vi "Digital_Input_Output_Ex.vi"() -> ()   [LabVIEW 2026]
panel:
  in  "Canal Read":u8
  out "Out":bool
  in  "VISA resource name":refnum<visa-resource-name>
  in  "Canal Write":u8
  out "respuesta":string
  in  "Stop Button":bool
  out "error out":errorcluster
  # "Ejemplo: Digital Input Output"
  # "Descripción: Lee un pin digital de entrada y escribe su estado en un pin de salida del microcontrolador."
  # "Configuracion"
  # "Indicadores"
  # "Control"
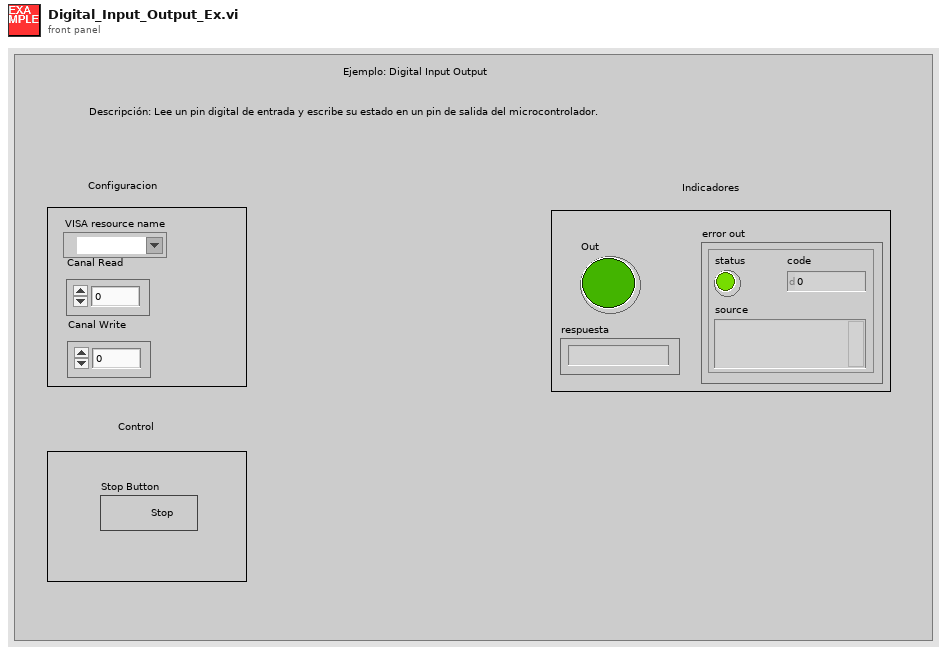
[diagram p1: front panel]
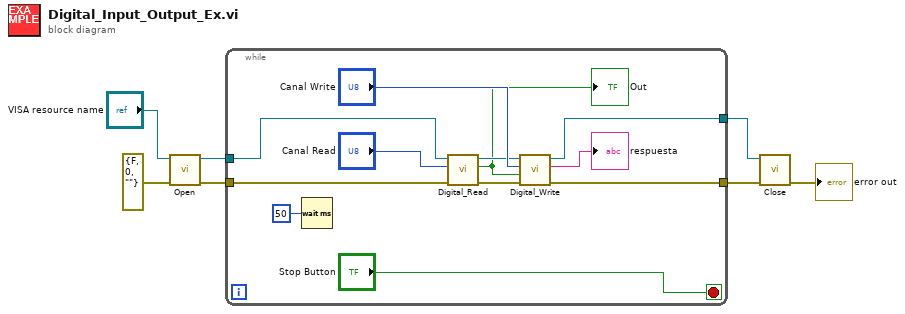
[diagram p0: block diagram]
diagram:
  n1 = call "Open.vi"("error in (no error)"=errorcluster {"status"=FALSE, "code"=0, "source"=""}, "VISA resource name"="VISA resource name") -> ("error out"=w7:errorcluster, "VISA resource name out"=w1:refnum<visa-resource-name>)  [unwired: 8 in]
  n2 = while {
    tunnel: [w16] -> w6
    tunnel: w7 -> [w12]
    tunnel: [w18] -> w5
    tunnel: w1 -> [w13]
    stop <- "Stop Button" stop-if-true
    n3 = Wait (ms)(milliseconds to wait=u32 50) -> ()  [unwired: 1 out]
    n4 = call "Digital_Read.vi"("error in (no error)"=w12, "Canal"="Canal Read", "VISA resource name"=w13) -> ("error out"=w11:errorcluster, "Out"=w10:bool, "VISA resource name out"=w14:refnum<visa-resource-name>)  [unwired: 6 in]
    "Out" <- w10
    n5 = call "Digital_Write.vi"("error in (no error)"=w11, "Valor"=w10, "Canal"="Canal Write", "VISA resource name"=w14) -> ("error out"=w18:errorcluster, "respuesta"=→"respuesta":string, "VISA resource name out"=w16:refnum<visa-resource-name>)  [unwired: 5 in]
  }
  n6 = call "Close.vi"("error in (no error)"=w5, "VISA resource name"=w6) -> ("error out"=→"error out":errorcluster)  [unwired: 9 in]
